vi "To String.vi"(8 "error in (no error)":errorcluster, 11 "Double Float in":refnum<class "Abs_Time 1D.lvclass">) -> (0 "error out":errorcluster, 2 "String":string, 3 "Double Float out":refnum<class "Abs_Time 1D.lvclass">)   [LabVIEW 2021, in "Abs_Time 1D.lvclass"]
uses:
  Abs_Time 1D.lvclass
  C:/TSA/LV_Abstract/Source/Abs_Types/Numeric 1D/Abs_Numeric_1D.lvclass
  Numeric 1D/Abs_Numeric_1D.lvclass/Abs_Numeric_1D.ctl
  Abs_Time 1D.lvclass/Abs_Time 1D.ctl
  Numeric 1D/Properties/Read Units.vi
  Properties/Read UTC Time For String Format.vi
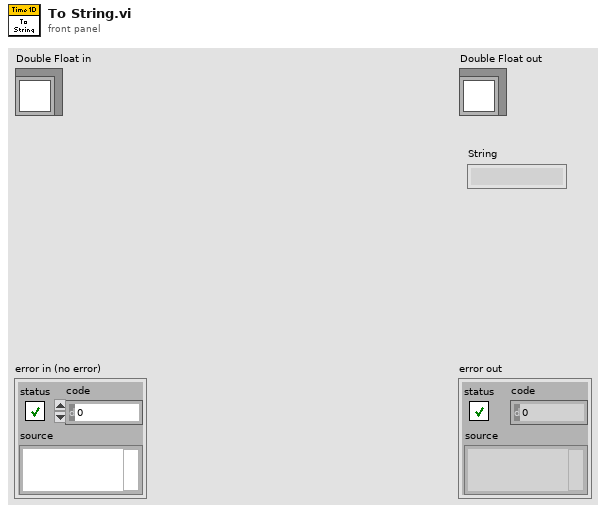
[diagram p1: front panel]
types:
  T1 = typedef "Abs_Time 1D.lvclass/Type.ctl" = timestamp[]
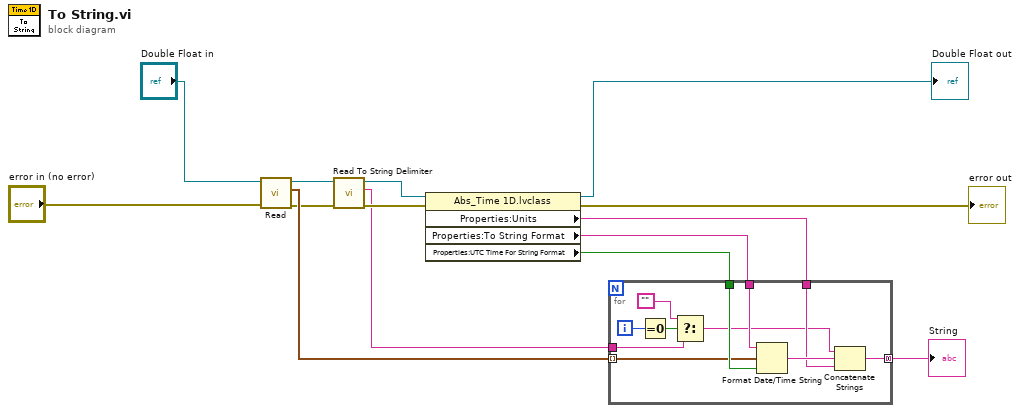
[diagram p0: block diagram]
diagram:
  n1 = call-dynamic "Read.vi"("error in (no error)"="error in (no error)", "Double Float.lvclass_340760 in"="Double Float in") -> ("error out"=w4:errorcluster, "Value"=w6:T1, "Double Float.lvclass_340760 out"=w5:refnum<class "Abs_Time 1D.lvclass">)  [unwired: 7 in]
  n2 = call-dynamic "Read To String Delimiter.vi"("error in (no error)"=w4, "Abs_Time 1D in"=w5) -> ("error out"=w3:errorcluster, "Delimiter"=w1:string, "Abs_Time 1D out"=w2:refnum<class "Abs_Time 1D.lvclass">)  [unwired: 7 in]
  n3 = property class="Abs_Time 1D.lvclass"(reference=w2, error in=w3) -> (reference out=→"Double Float out":refnum<class "Abs_Time 1D.lvclass">, error out=→"error out":errorcluster, "Properties:Units"=w7:string, "Properties:To String Format"=w9:string, "Properties:UTC Time For String Format"=w8:bool)
  n4 = for {
    tunnel: w8 -> [w22]
    tunnel: w7 -> [w21]
    tunnel: w9 -> [w23]
    tunnel: [w25] -> w13 mode=concatenating
    tunnel: w6 -> [w20] mode=indexing
    tunnel: w1 -> [w15]
    i -> [w19]
    n5 = Equal To 0?(x=w19) -> (x = 0?=w18:bool)
    n6 = Select(t="", s=w18, f=w15) -> (s? t:f=w16:string)
    n7 = Format Date/Time String(time format string (%c)=w23, seconds (now)=w20, UTC format=w22) -> (date/time string=w24:string)
    n8 = Concatenate Strings(w16, w24, w21) -> (w25:string)
  }
  "String" <- w13
